vi "syd-PhasicFunctionv2.vi"() -> ()   [LabVIEW 2026]
uses:
  <vilib>/DAQmx/read.llb/DAQmx Read (Analog 1D Wfm NChan NSamp).vi
  <vilib>/DAQmx/create/channels.llb/DAQmx Create Channel (AI-Voltage-Basic).vi
  <vilib>/DAQmx/configure/timing.llb/DAQmx Timing (Sample Clock).vi
  <vilib>/DAQmx/miscellaneous.llb/DAQmx Fill In Error Info.vi
panel:
  in  "test duration (min)":dbl
  out "Waveform Chart":waveform(dbl)[](graph)
  in  "error in":errorcluster
  out "data 2":waveform(dbl)[](graph) caption="data"
  in  "stop 2":bool caption="stop"
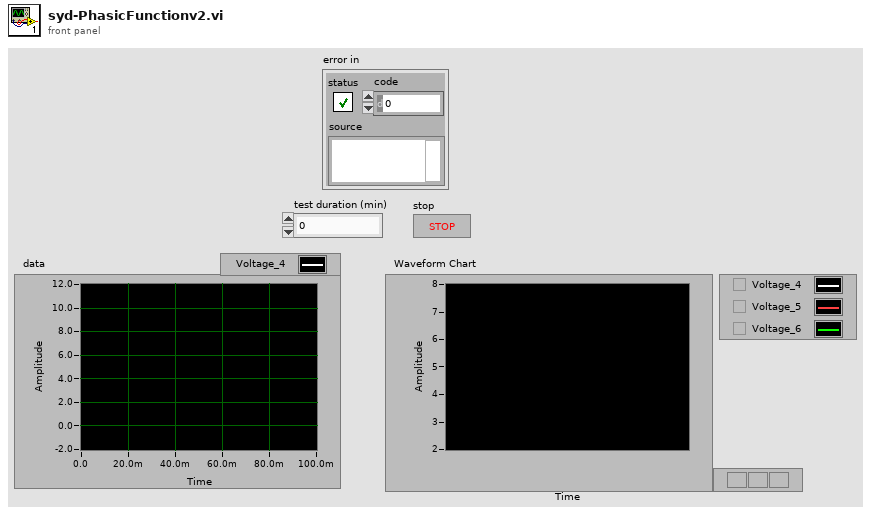
[diagram p1: front panel]
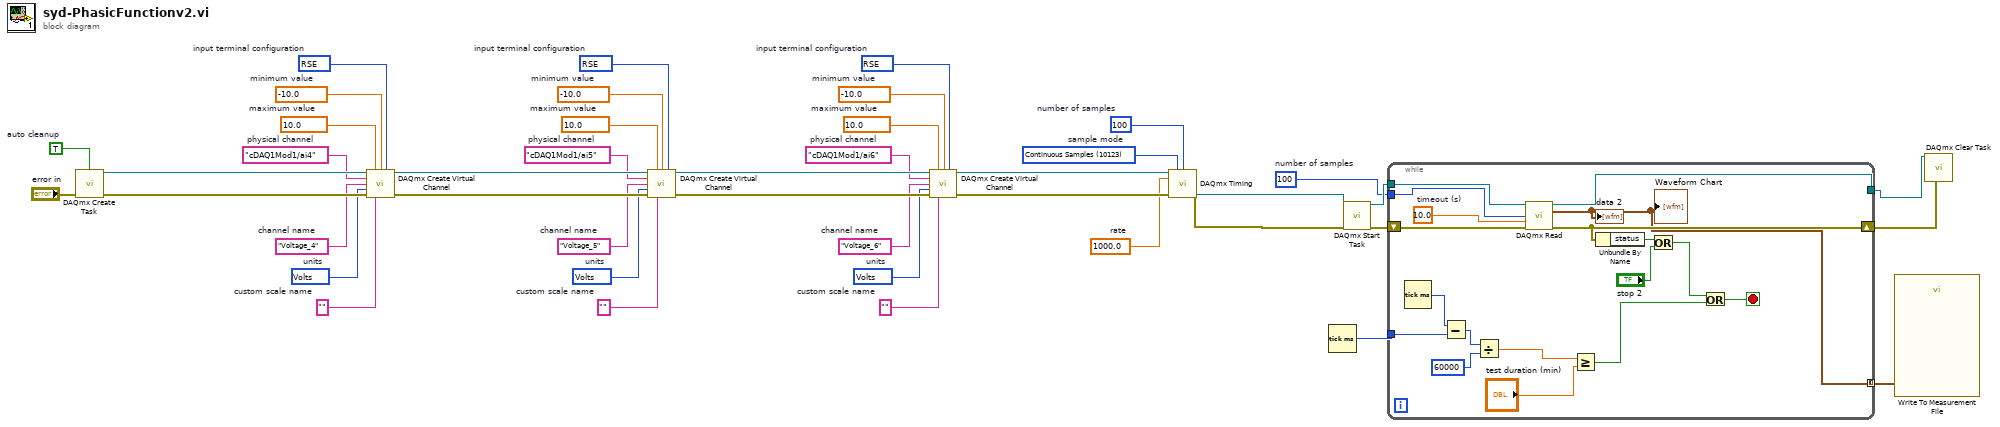
[diagram p0: block diagram]
diagram:
  w5 = 10123 items=["Finite Samples"=10178, "Continuous Samples"=10123, "Hardware Timed Single Point"=12522]  # sample mode
  w6 = 100  # number of samples
  w7 = 1000.0  # rate
  w9 = 10083 items=["default"=-1, "RSE"=10083, "NRSE"=10078, "Differential"=10106, "Pseudodifferential"=12529]  # input terminal configuration
  w10 = 10348 items=["Volts"=10348, "From Custom Scale"=10065]  # units
  w11 = "Voltage_6"  # channel name
  w13 = ""  # custom scale name
  w14 = -10.0  # minimum value
  w15 = 10.0  # maximum value
  w16 = "cDAQ1Mod1/ai6"  # physical channel
  w18 = 10083 items=["default"=-1, "RSE"=10083, "NRSE"=10078, "Differential"=10106, "Pseudodifferential"=12529]  # input terminal configuration
  w19 = 10348 items=["Volts"=10348, "From Custom Scale"=10065]  # units
  w20 = "Voltage_5"  # channel name
  w22 = ""  # custom scale name
  w23 = -10.0  # minimum value
  w24 = 10.0  # maximum value
  w25 = "cDAQ1Mod1/ai5"  # physical channel
  w27 = 10083 items=["default"=-1, "RSE"=10083, "NRSE"=10078, "Differential"=10106, "Pseudodifferential"=12529]  # input terminal configuration
  w28 = 10348 items=["Volts"=10348, "From Custom Scale"=10065]  # units
  w29 = "Voltage_4"  # channel name
  w31 = ""  # custom scale name
  w32 = -10.0  # minimum value
  w33 = 10.0  # maximum value
  w34 = "cDAQ1Mod1/ai4"  # physical channel
  w36 = TRUE  # auto cleanup
  w41 = 100  # number of samples
  n1 = call <vilib>:"DAQmx Create Task.vi"("auto cleanup"=w36, "error in"="error in") -> ("task out"=w35:refnum<k21>, "error out"=w37:errorcluster)  [unwired: 12 in]
  n2 = call-poly <vilib>:"DAQmx Create Virtual Channel.vi"("task in"=w35, "maximum value"=w33, "minimum value"=w32, "input terminal configuration"=w27, "physical channels"=w34, "name to assign"=w29, "units"=w28, "error in"=w37, "custom scale name"=w31) -> ("task out"=w26:refnum<k21>, "error out"=w30:errorcluster)  [unwired: 5 in]
  n3 = call-poly <vilib>:"DAQmx Create Virtual Channel.vi"("task in"=w26, "maximum value"=w24, "minimum value"=w23, "input terminal configuration"=w18, "physical channels"=w25, "name to assign"=w20, "units"=w19, "error in"=w30, "custom scale name"=w22) -> ("task out"=w17:refnum<k21>, "error out"=w21:errorcluster)  [unwired: 5 in]
  n4 = call-poly <vilib>:"DAQmx Create Virtual Channel.vi"("task in"=w17, "maximum value"=w15, "minimum value"=w14, "input terminal configuration"=w9, "physical channels"=w16, "name to assign"=w11, "units"=w10, "error in"=w21, "custom scale name"=w13) -> ("task out"=w8:refnum<k21>, "error out"=w12:errorcluster)  [unwired: 5 in]
  n5 = call-poly <vilib>:"DAQmx Timing.vi"("task/channels in"=w8, "sample mode"=w5, "samples per channel"=w6, "rate"=w7, "error in"=w12) -> ("task out"=w3:refnum<k21>, "error out"=w4:errorcluster)  [unwired: 9 in]
  n6 = Tick Count (ms)() -> (millisecond timer value=w1:u32)
  n7 = call <vilib>:"DAQmx Start Task.vi"("task/channels in"=w3, "error in"=w4) -> ("task out"=w43:refnum<k21>, "error out"=w42:errorcluster)  [unwired: 12 in]
  n8 = while {
    tunnel: w43 -> [w61]
    tunnel: w41 -> [w58]
    tunnel: [w59] -> w39
    shift-right: [w56] -> w40
    shift-left: w42 -> [w60]
    tunnel: [w53] -> w2 mode=concatenating
    tunnel: w1 -> [w52]
    stop <- w44 stop-if-true
    w54 = 10.0  # timeout (s)
    n9 = Tick Count (ms)() -> (millisecond timer value=w51:u32)
    n10 = Subtract(x=w51, y=w52) -> (x-y=w50:u32)
    n11 = Divide(x=w50, y=60000) -> (x/y=w48:dbl)
    n12 = call-poly <vilib>:"DAQmx Read.vi"("task/channels in"=w61, "number of samples per channel"=w58, "timeout"=w54, "error in"=w60) -> ("task out"=w59:refnum<k21>, "data"=w53:waveform(dbl)[], "error out"=w56:errorcluster)  [unwired: 9 in]
    "data 2" <- w53
    "Waveform Chart" <- w53
    n13 = Greater Or Equal?(x=w48, y="test duration (min)") -> (x >= y?=w46:bool)
    n14 = Unbundle By Name(w56) -> ("status"=w57:bool)
    n15 = Or(x=w57, y="stop 2") -> (x .or. y?=w45:bool)
    n16 = Or(x=w45, y=w46) -> (x .or. y?=w44:bool)
  }
  n17 = call "Write To Measurement File"("Signals"=w2) -> ()  [unwired: 16 in, 3 out]
  n18 = call <vilib>:"DAQmx Clear Task.vi"("task in"=w39, "error in"=w40) -> ()  [unwired: 13 in, 1 out]
